vi "Boite Dialogue 2 boutons.vi"(1 "bouton droit visible ?":bool, 2 "Texte bouton droit":string, 3 "Texte bouton gauche":string, 4 "Message":string) -> (0 "Bouton droit ?":bool)   [LabVIEW 2022 SP3]
panel:
  in  "Bouton gauche":bool
  in  "Bouton droit":bool
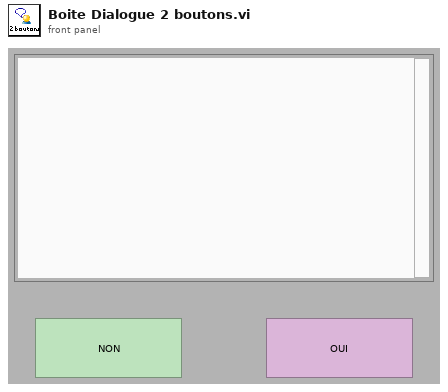
[diagram p1: front panel]
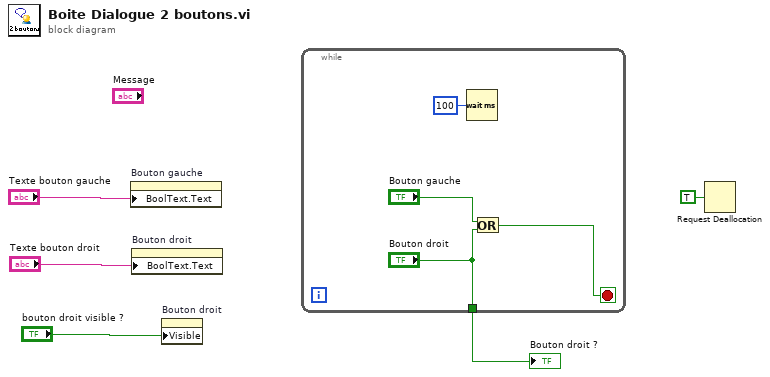
[diagram p0: block diagram]
diagram:
  n1 = property on="Bouton gauche" class="Bool"("BoolText.Text"="Texte bouton gauche") -> ()  [unwired: 2 in, 2 out]
  n2 = property on="Bouton droit" class="Bool"("BoolText.Text"="Texte bouton droit") -> ()  [unwired: 2 in, 2 out]
  n3 = property on="Bouton droit" class="Bool"("Visible"="bouton droit visible ?") -> ()  [unwired: 2 in, 2 out]
  n4 = while {
    tunnel: ["Bouton droit"] -> w5
    stop <- w8 stop-if-true
    n5 = Wait (ms)(milliseconds to wait=u32 100 ("attente (ms)")) -> ()  [unwired: 1 out]
    n6 = Or(x="Bouton gauche", y="Bouton droit") -> (x .or. y?=w8:bool)
  }
  "Bouton droit ?" <- w5
  n7 = Request Deallocation(TRUE ("flag")) -> ()
